vi "Capture_Loop.vi"(8 "error in (no error)":errorcluster={"status"=FALSE, "code"=0, "source"="\"\""}, 10 "sample stream":string, 11 "CaptureRequest queue":string) -> (0 "error out":errorcluster={"status"=FALSE, "code"=0, "source"="\"\""}, 2 "status ok":bool, 3 "CaptureStatus/results":string)   [LabVIEW 2026]
doc: "INTENT: Own measurement capture service. LOGIC: Schedule sessions, aggregate timestamped samples, finalize on sample/time condition or interruption."
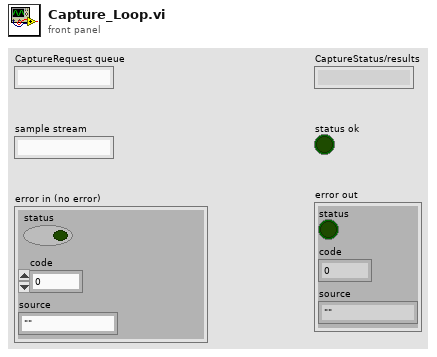
[diagram p1: front panel]
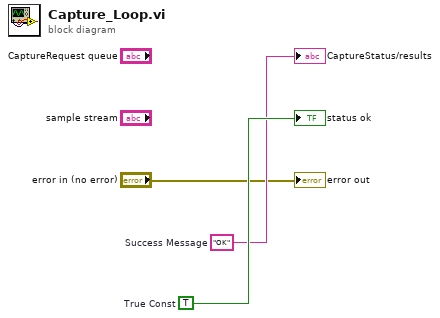
[diagram p0: block diagram]
diagram:
  w3 = TRUE  # True Const
  w2 = "OK"  # Success Message
  "CaptureStatus/results" <- w2
  "status ok" <- w3
  "error out" <- "error in (no error)"
